vi "Resolve Template Value.vi"(6 "Locals":refnum<class "Value Tree.lvclass">, 7 "Folder":path, 8 "error in (no error)":errorcluster, 9 "Template Service in":refnum<class "TemplateService.lvclass">, 10 "Value Name":string, 11 "TemplateVariableResolver in":refnum<class "TemplateValueResolver.lvclass">) -> (0 "error out":errorcluster, 1 "Template Service":refnum<class "TemplateService.lvclass">, 2 "Value":refnum<class "Value Tree.lvclass">)   [LabVIEW 2020, in "HTTP Server.lvlib" / "TemplateValueResolver.lvclass"]
uses:
  TemplateValueResolver.lvclass
  Value Tree/Value Tree.lvclass
  TemplateService/TemplateService.lvclass
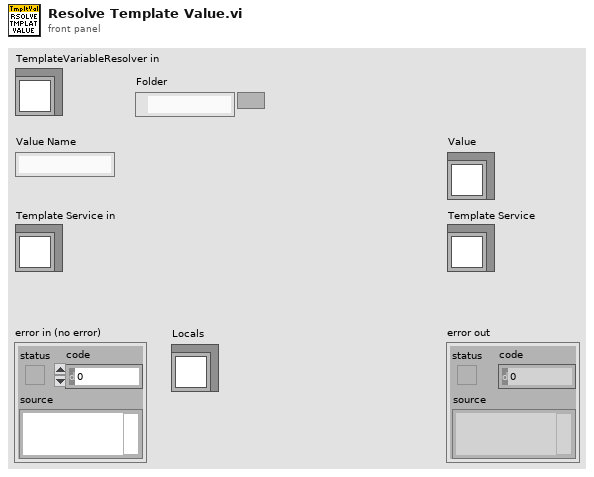
[diagram p1: front panel]
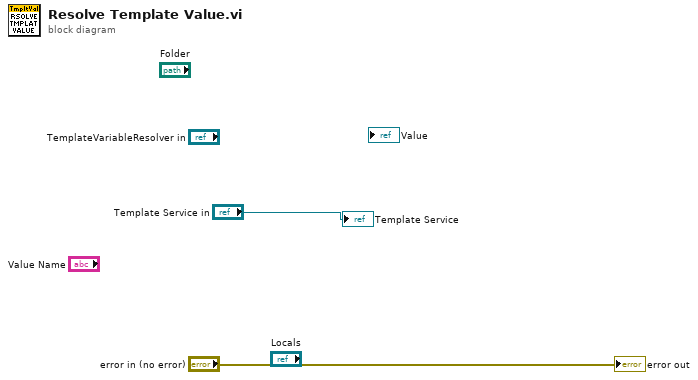
[diagram p0: block diagram]
diagram:
  "error out" <- "error in (no error)"
  "Template Service" <- "Template Service in"
